vi "AR table formation VI.vi"(8 "AA2 info":T1, 9 "A Cluster":T4, 10 "AA info":T2, 11 "info Cluster":T3) -> (3 "AR Table Data":string[](array[string]))   [LabVIEW 2018]
panel:
  out "Selection":enum16{"10kHz", "100kHz"}(ring)
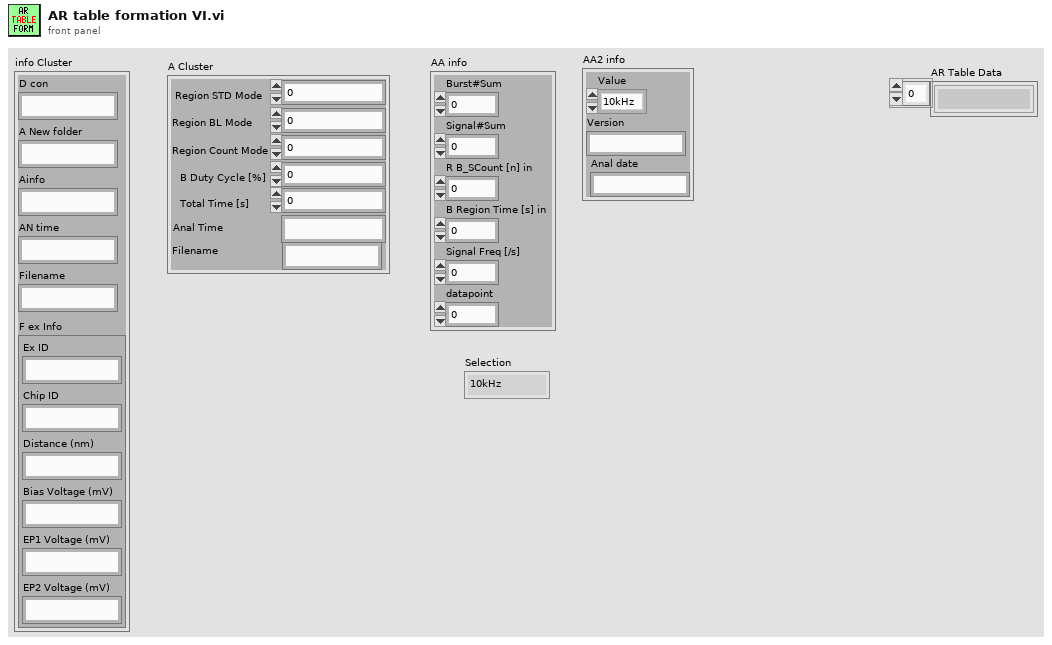
[diagram p1: front panel]
types:
  T1 = cluster{"Value":enum16{"10kHz", "100kHz"}, "Version":string, "Anal date":string}
  T2 = cluster{"Burst#Sum":i32, "Signal#Sum":i32, "R B_SCount [n] in":i32, "B Region Time [s] in":dbl, "Signal Freq [/s]":dbl, "datapoint":i32}
  T3 = cluster{"D con":string, "A New folder":string, "Ainfo":string, "AN time":string, "Filename":string, "F ex Info":cluster{"Ex ID":string, "Chip ID":string, "Distance (nm)":string, "Bias Voltage (mV)":string, "EP1 Voltage (mV)":string, "EP2 Voltage (mV)":string}}
  T4 = cluster{"Region STD Mode":dbl, "Region BL Mode":dbl, "Region Count Mode":dbl, "B Duty Cycle [%]":dbl, "Total Time [s]":dbl, "Anal Time":string, "Filename":string}
  T5 = cluster{"Ex ID":string, "Chip ID":string, "Distance (nm)":string, "Bias Voltage (mV)":string, "EP1 Voltage (mV)":string, "EP2 Voltage (mV)":string}
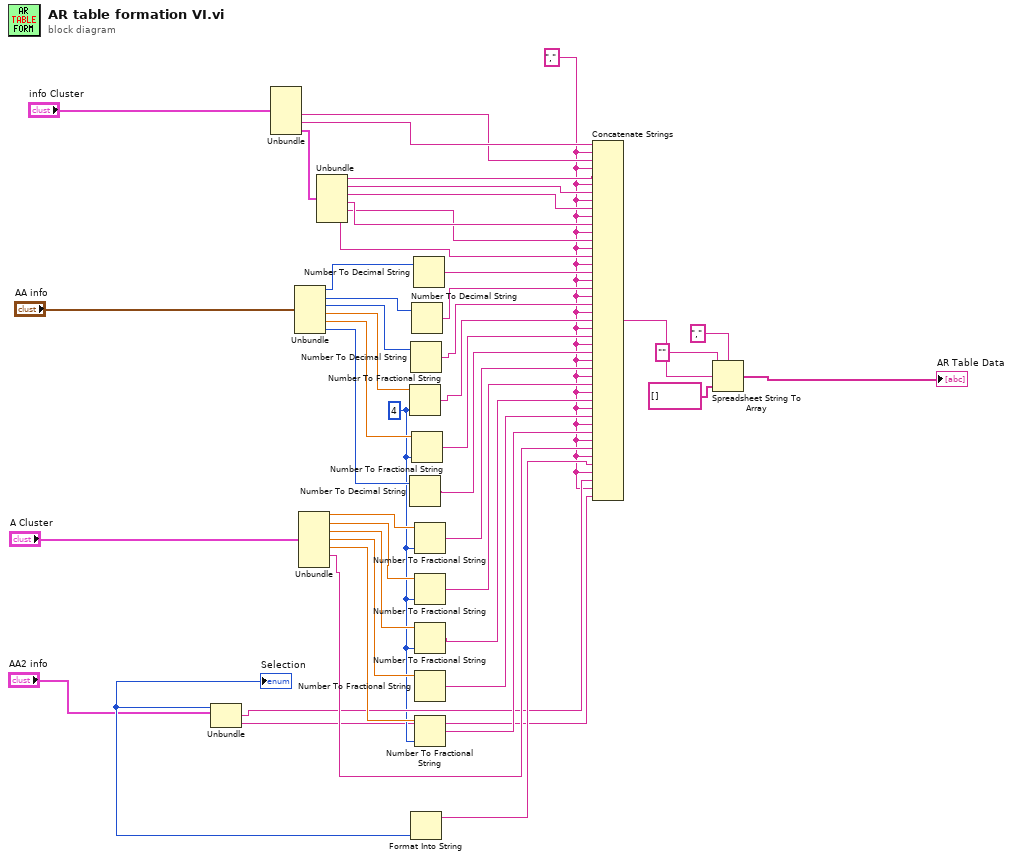
[diagram p0: block diagram]
diagram:
  w4 = i16 4 ("精度（6）")
  w2 = "," ("デリミタ（タブ）")
  n1 = Unbundle("AA2 info") -> ("Value"=w6:enum16{"10kHz", "100kHz"}, "Version"=w5:string, "Anal date"=w1:string)
  "Selection" <- w6
  n2 = Unbundle("info Cluster") -> ("AN time"=w24:string, "Filename"=w25:string, "F ex Info"=w26:T5)  [unwired: 3 out]
  n3 = Unbundle("AA info") -> ("Burst#Sum"=w35:i32, "Signal#Sum"=w34:i32, "R B_SCount [n] in"=w33:i32, "B Region Time [s] in"=w31:dbl, "Signal Freq [/s]"=w29:dbl, "datapoint"=w19:i32)
  n4 = Unbundle("A Cluster") -> ("Region STD Mode"=w15:dbl, "Region BL Mode"=w14:dbl, "Region Count Mode"=w12:dbl, "B Duty Cycle [%]"=w11:dbl, "Total Time [s]"=w10:dbl, "Anal Time"=w9:string)  [unwired: 1 out]
  n5 = Unbundle(w26) -> ("Ex ID"=w23:string, "Chip ID"=w22:string, "Distance (nm)"=w21:string, "Bias Voltage (mV)"=w18:string, "EP1 Voltage (mV)"=w17:string, "EP2 Voltage (mV)"=w16:string)
  n6 = Number To Fractional String(number=w31, precision (6)=w4) -> (F-format string=w30:string)  [unwired: 2 in]
  n7 = Number To Decimal String(number=w19) -> (decimal integer string=w28:string)  [unwired: 1 in]
  n8 = Number To Decimal String(number=w33) -> (decimal integer string=w32:string)  [unwired: 1 in]
  n9 = Format Into String(w6) -> (resulting string=w8:string)  [unwired: 3 in, 1 out]
  n10 = Number To Decimal String(number=w34) -> (decimal integer string=w46:string)  [unwired: 1 in]
  n11 = Number To Fractional String(number=w29, precision (6)=w4) -> (F-format string=w45:string)  [unwired: 2 in]
  n12 = Number To Decimal String(number=w35) -> (decimal integer string=w47:string)  [unwired: 1 in]
  n13 = Number To Fractional String(number=w15, precision (6)=w4) -> (F-format string=w44:string)  [unwired: 2 in]
  n14 = Number To Fractional String(number=w14, precision (6)=w4) -> (F-format string=w43:string)  [unwired: 2 in]
  n15 = Number To Fractional String(number=w12, precision (6)=w4) -> (F-format string=w13:string)  [unwired: 2 in]
  n16 = Number To Fractional String(number=w11) -> (F-format string=w42:string)  [unwired: 3 in]
  n17 = Number To Fractional String(number=w10, precision (6)=w4) -> (F-format string=w41:string)  [unwired: 2 in]
  n18 = Concatenate Strings(w25, w2, w24, w2, w23, w2, w22, w2, w21, w2, w18, w2, w17, w2, w16, w2, w47, w2, w46, w2, w32, w2, w30, w2, w45, w2, w28, w2, w44, w2, w43, w2, w13, w2, w42, w2, w41, w2, w9, w2, w8, w2, w5, w2, w1) -> (w37:string)
  n19 = Spreadsheet String To Array(delimiter (Tab)="," ("デリミタ（タブ）"), format string="" ("形式文字列"), spreadsheet string=w37, array type (2D Dbl)=string[] [] ("行ヘッダ文字列[]")) -> (array=→"AR Table Data":string[])
